vi "Check Queue Count.vi"() -> ()   [LabVIEW 2020]
doc: "Enqueue 50 messages and use inspection tool to get message count\nensure count matches the number of queued messages"
uses:
  ActorFramework/Actor/Actor.lvclass
  ActorFramework/Message/Message.lvclass
  ActorFramework/Message Queue/Message Queue.lvclass/Message Queue.ctl
  ActorFramework/Message Enqueuer/Message Enqueuer.lvclass/Message Enqueuer.ctl
  ActorFramework/Stop Msg/Stop Msg.lvclass
  C:/Users/Neil/Documents/actor-framework/Core/ActorFramework/Message/Message.lvclass
  ActorFramework/Message Priority Queue/Priority Enqueue.vi
  <vilib>/addons/_JKI Toolkits/Caraya/classes/Assert/Assert Equal Value_Variant.vi
  <vilib>/addons/_JKI Toolkits/Caraya/classes/Test/Test.lvclass
  <vilib>/addons/_JKI Toolkits/Caraya/classes/Assert/Assert.lvclass
  ActorFramework/Message Queue/Message Queue.lvclass
  ActorFramework/Message Enqueuer/Message Enqueuer.lvclass
panel:
  out "# elements in queue":i32
  out "Element Names":string[](array[string])
  out "error out":errorcluster
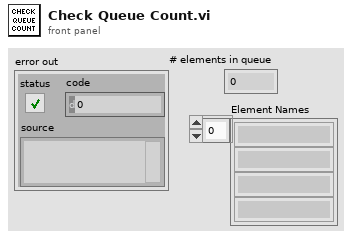
[diagram p1: front panel]
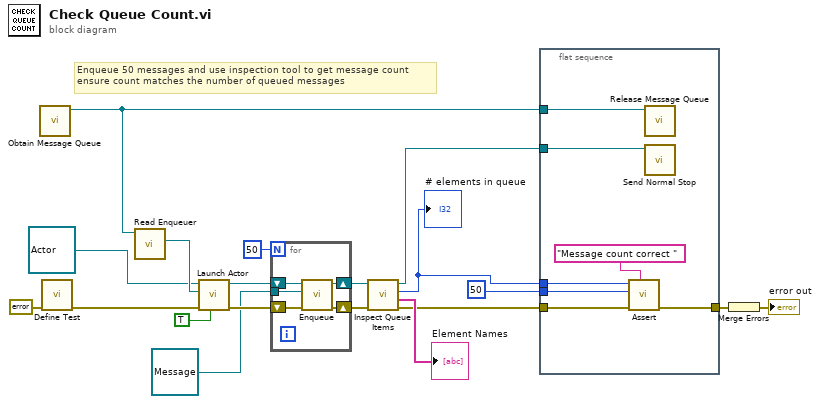
[diagram p0: block diagram]
diagram:
  # "Enqueue 50 messages and use inspection tool to get message count\nensure count matches the number of queued messages"
  n1 = call "Obtain Message Queue.vi"() -> ("Message Queue"=w14:refnum<class "Message Queue.lvclass">)  [unwired: 10 in, 1 out]
  n2 = call <vilib>:"Define Test.vi"("error in (no error)"=errorcluster {"status"=FALSE, "code"=0, "source"=""}) -> ("error out"=w17:errorcluster)  [unwired: 9 in, 1 out]
  n3 = call "Read Enqueuer.vi"("Message Queue"=w14) -> ("Message Enqueuer"=w16:refnum<class "Message Enqueuer.lvclass">)  [unwired: 10 in]
  n4 = call "Launch Actor.vi"("Open Actor Core front panel? (F)"=TRUE, "error in (no error)"=w17, "Actor-to-Caller Enqueuer"=w16, "Actor"=refnum<class "Actor.lvclass"> refnum) -> ("error out"=w9:errorcluster, "Caller-To-Actor Enqueuer"=w10:refnum<class "Message Enqueuer.lvclass">)  [unwired: 6 in]
  n5 = for {
    N: 50 -> [_]
    tunnel: refnum<class "Message.lvclass"> refnum ("Message") -> [w22]
    shift-right: [w21] -> w3
    shift-left: w10 -> [w24]
    shift-right: [w20] -> w2
    shift-left: w9 -> [w23]
    n6 = call "Enqueue.vi"("error in (no error)"=w23, "Message"=w22, "Message Enqueuer in"=w24) -> ("error out"=w20:errorcluster, "Message Enqueuer out"=w21:refnum<class "Message Enqueuer.lvclass">)  [unwired: 7 in]
  }
  n7 = call "Inspect Queue Items.vi"("error in (no error)"=w2, "Message Enqueuer in"=w3) -> ("error out"=w5:errorcluster, "Element Names"=→"Element Names":string[], "# elements in queue"=w4:i32, "Message Enqueuer out"=w6:refnum<class "Message Enqueuer.lvclass">)  [unwired: 6 in]
  "# elements in queue" <- w4
  n8 = flat-sequence {
    tunnel: [w30] -> w19
    tunnel: w5 -> [w29]
    tunnel: w14 -> [w28]
    tunnel: w4 -> [w27]
    tunnel: 50 -> [w26]
    tunnel: w6 -> [w25]
    frame #0 {
      n9 = call-poly <vilib>:"Assert.vi"("Label"="Message count correct " ("Label (VI Title)"), "error in (no error)"=w29, "Actual"=w26, "Expected"=w27) -> ("error out"=w30:errorcluster)  [unwired: 6 in, 1 out]
      n10 = call "Release Message Queue.vi"("Message Queue"=w28) -> ()  [unwired: 9 in, 2 out]
      n11 = call "Send Normal Stop.vi"("Message Enqueuer"=w25) -> ()  [unwired: 10 in, 1 out]
    }
  }
  n12 = Merge Errors(w19) -> (→"error out":errorcluster)
